vi "VIH HelpGen - Get Control Terminal Image - Temp VI Refnum.vi"(6 "cmd (get)":enum16{"get", "close"}(ring), 8 "error in":errorcluster) -> (0 "error out":errorcluster, 3 "VI Refnum":refnum<vi>)   [LabVIEW 2014]
doc: "::: VI Helpeks :::\nCopyright (c) 2000-2026 Konstantin Shifershteyn. All rights reserved."
panel:
  # "VI Helpeks\nCopyright (c) 2012-2026 Konstantin Shifershteyn"
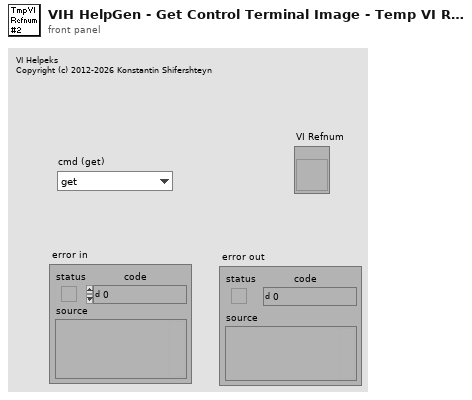
[diagram p1: front panel]
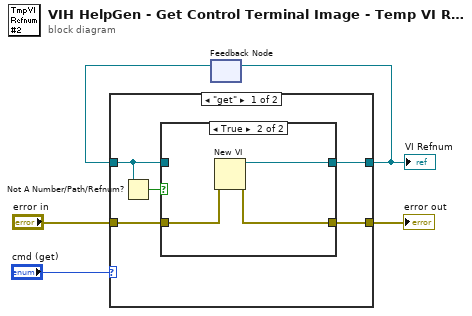
[diagram p0: block diagram]
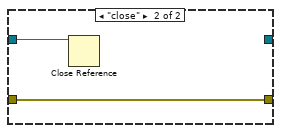
[diagram p3: hidden frame]
diagram:
  n1 = feedback #1() -> (w4:refnum<vi>)  [unwired: 1 in]
  n2 = case shown="\"get\"" "cmd (get)" {
    tunnel: [w10 _] -> w5
    tunnel: w4 -> [w9 w17]
    tunnel: "error in" -> [w7 w16]
    tunnel: [w6 w16] -> w1
    frame "get" {
      n3 = Not A Number/Path/Refnum?(number/path/refnum=w9) -> (NaN/Path/Refnum?=w8:bool)
      n4 = case shown="True" w8 {
        tunnel: [w12 w15] -> w10
        tunnel: w9 -> [w12 _]
        tunnel: w7 -> [w11 w14]
        tunnel: [w11 w13] -> w6
        frame False {
        }
        frame True {
          n5 = New VI(8:w14) -> (0:w13:errorcluster, 3:w15:refnum<vi>)  [unwired: 6 in]
        }
      }
    }
    frame "close" {
      n6 = Close Reference(reference=w17) -> ()  [unwired: 1 in, 1 out]
    }
  }
  "error out" <- w1
  "VI Refnum" <- w5
  n7 = feedback-in #1(w5) -> ()
